vi "Apply Style - Simple Dialog.vi"(4 "button refs":refnum<vi>[](array[refnum]), 6 "keep transparent buttons?":bool, 7 "title ref":refnum<vi>, 8 "error in":errorcluster, 9 "message ref":refnum<vi>, 10 "pop up ref":refnum<vi>, 11 "Theme in":refnum<class "Theme.lvclass">) -> (0 "error out":errorcluster, 3 "Theme out":refnum<class "Theme.lvclass">)   [LabVIEW 2021, in "Theme.lvclass"]
doc: "Apply the style to the message pop up : format the header, background, and message box\n\n<b>Code Developed By:</b> +\nDaniel Coons +\nhttps://github.com/danielcoons/tsc-pop-up"
uses:
  Theme.lvclass
  <vilib>/Utility/miscctls.llb/LVSelectionTypeDef.ctl
  Theme.lvclass/Theme.ctl
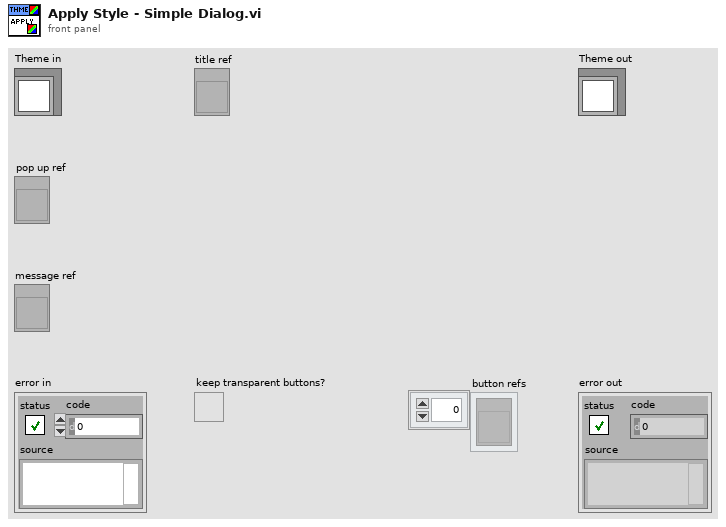
[diagram p1: front panel]
types:
  T1 = typedef "LVSelectionTypeDef.ctl" = cluster{"Selection Start":u32, "Selection End":u32}
  T2 = typedef "Theme.lvclass/Button colors--typedef.ctl" = cluster{"false color":cluster{"border":u32, "fill":u32}, "hover color":cluster{"border":u32, "fill":u32}, "press color":cluster{"border":u32, "fill":u32}, "Boolean Text":u32, "Text.Font Name":string, "Text.Font Size":u32, "Bold?":bool, "Itallic?":bool}
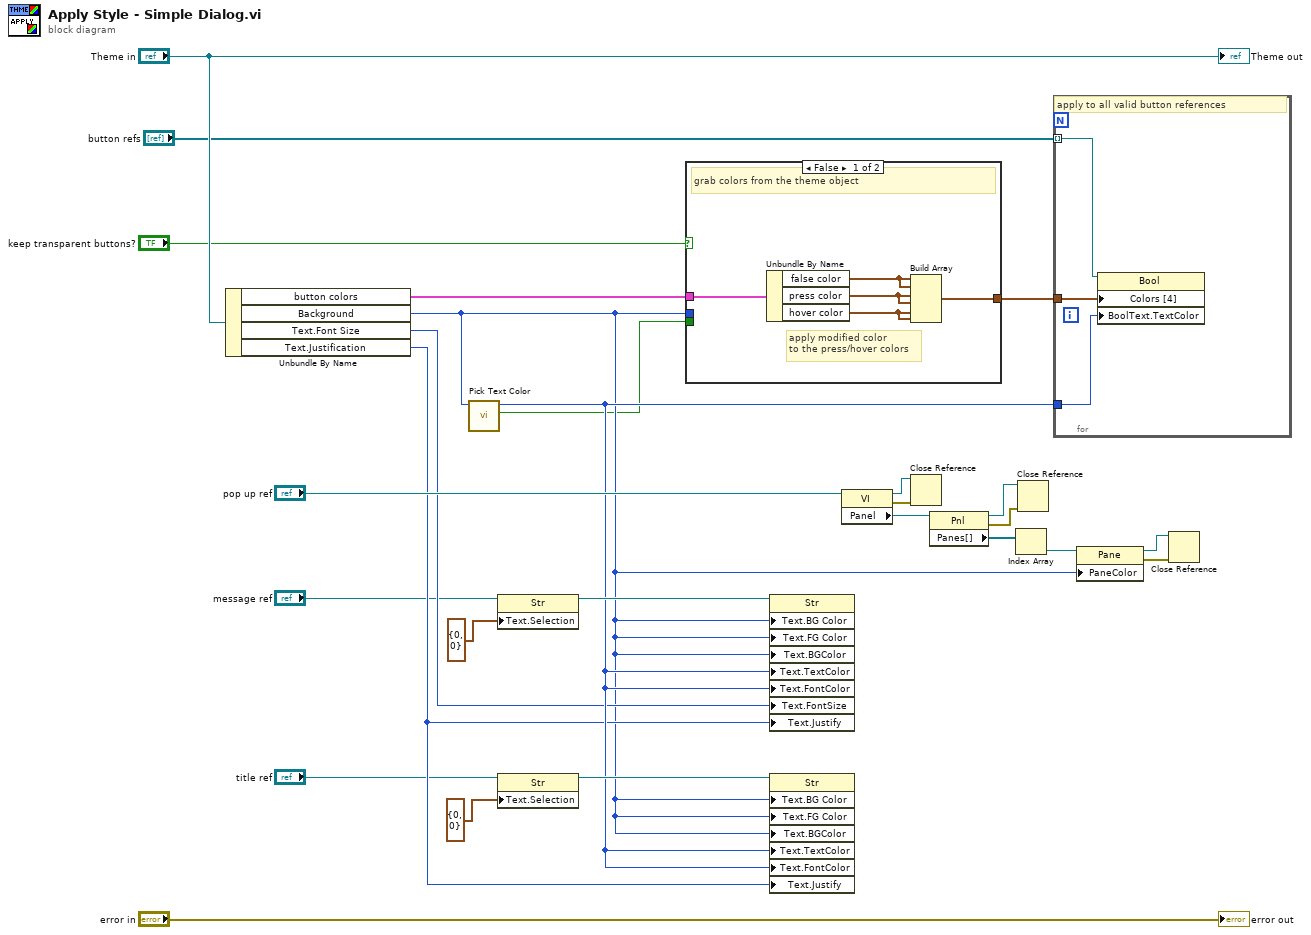
[diagram p0: block diagram]
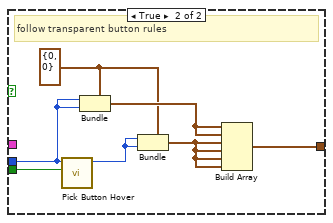
[diagram p2: hidden frame]
diagram:
  n1 = Unbundle By Name("Theme in") -> ("button colors"=w2:T2, "Background"=w5:u32, "Text.Font Size"=w9:u32, "Text.Justification"=w8:enum16{"Left", "Center", "Right"})
  n2 = call "Pick Text Color.vi"("color"=w5) -> ("light?"=w4:bool, "text"=w10:u32)  [unwired: 9 in]
  n3 = property class="Str"(reference="message ref", "Text.Selection"=T1 {"Selection Start"=0, "Selection End"=0}) -> (reference out=w14:refnum<vi>)  [unwired: 1 in, 1 out]
  n4 = property class="Str"(reference="title ref", "Text.Selection"=T1 {"Selection Start"=0, "Selection End"=0}) -> (reference out=w11:refnum<vi>)  [unwired: 1 in, 1 out]
  n5 = case shown="False" "keep transparent buttons?" {
    tunnel: w5 -> [_ w38]
    tunnel: w4 -> [_ w39]
    tunnel: w2 -> [w32 _]
    tunnel: [w28 w33] -> w1
    frame False {
      # "apply modified color \nto the press/hover colors"
      # "grab colors from the theme object"
      n6 = Unbundle By Name(w32) -> ("false color"=w31:cluster{"border":u32, "fill":u32}, "press color"=w30:cluster{"border":u32, "fill":u32}, "hover color"=w29:cluster{"border":u32, "fill":u32})
      n7 = Build Array(w31, w31, w30, w30, w29, w29) -> (w28:cluster{"border":u32, "fill":u32}[])
    }
    frame True {
      w34 = cluster{u32, u32} {0, 0}
      # "follow transparent button rules"
      n8 = call "Pick Button Hover.vi"("light?"=w39, "Background"=w38) -> ("Color"=w37:u32)  [unwired: 9 in]
      n9 = Bundle(cluster=w34, w38, w38) -> (w35:cluster{u32, u32})
      n10 = Bundle(cluster=w34, w37, w37) -> (w36:cluster{u32, u32})
      n11 = Build Array(w35, w35, w36, w36, w36, w36) -> (w33:cluster{u32, u32}[])
    }
  }
  n12 = property on="Property Node" class="Str"(reference=w14, "Text.BG Color"=w5, "Text.FG Color"=w5, "Text.BGColor"=w5, "Text.TextColor"=w10, "Text.FontColor"=w10, "Text.FontSize"=w9, "Text.Justify"=w8) -> ()  [unwired: 1 in, 2 out]
  n13 = property on="Property Node" class="Str"(reference=w11, "Text.BG Color"=w5, "Text.FG Color"=w5, "Text.BGColor"=w5, "Text.TextColor"=w10, "Text.FontColor"=w10, "Text.Justify"=w8) -> ()  [unwired: 1 in, 2 out]
  n14 = property class="VI"(reference="pop up ref") -> (reference out=w16:refnum<vi>, error out=w24:errorcluster, "Panel"=w23:refnum<vi>)  [unwired: 1 in]
  n15 = Close Reference(reference=w16, error in (no error)=w24) -> ()  [unwired: 1 out]
  n16 = property class="Pnl"(reference=w23) -> (reference out=w17:refnum<vi>, error out=w25:errorcluster, "Panes[]"=w22:refnum<vi>[])  [unwired: 1 in]
  n17 = Index Array(array=w22) -> (element=w21:refnum<vi>)  [unwired: 1 in]
  n18 = Close Reference(reference=w17, error in (no error)=w25) -> ()  [unwired: 1 out]
  n19 = for {
    tunnel: "button refs" -> [w41] mode=indexing
    tunnel: w10 -> [w42]
    tunnel: w1 -> [w40]
    # "apply to all valid button references"
    n20 = property on="Property Node" class="Bool"(reference=w41, "Colors [4]"=w40, "BoolText.TextColor"=w42) -> ()  [unwired: 1 in, 2 out]
  }
  n21 = property class="Pane"(reference=w21, "PaneColor"=w5) -> (reference out=w18:refnum<vi>, error out=w26:errorcluster)  [unwired: 1 in]
  n22 = Close Reference(reference=w18, error in (no error)=w26) -> ()  [unwired: 1 out]
  "error out" <- "error in"
  "Theme out" <- "Theme in"
